vi "Spinner.vi"(5 "Enum":T1(ring)=enum."Spinner 4") -> (2 "Spinner Out":string="(---\\/------\\/---)")   [LabVIEW 2019, in "Instrument.Lockin.lvlib" / "Instrument UI.Lockin.lvclass"]
uses:
  Instrument UI.Lockin.lvclass
panel:
  in  "Spinner 6":string="(\\-\\-\\-----------)\n(-\\-\\-\\----------)\n(--\\-\\-\\---------)\n(---\\-\\-\\--------)\n(----\\-\\-\\-------)\n(-----\\-\\-\\------)\n(------\\-\\-\\-----)\n(-------\\-\\-\\----)\n(--------\\-\\-\\---)\n(---------\\-\\-\\--)\n(----------\\-\\-\\-)\n(-----------\\-\\-\\)\n(----------\\-\\-\\-)\n(---------\\-\\-\\--)\n(--------\\-\\-\\---)\n(-------\\-\\-\\----)\n(------\\-\\-\\-----)\n(-----\\-\\-\\------)\n(----\\-\\-\\-------)\n(---\\-\\-\\--------)\n(--\\-\\-\\---------)\n(-\\-\\-\\----------)"
  in  "Spinner 5":string="(\\------/\\------/)\n(-\\----/--\\----/-)\n(--\\--/----\\--/--)\n(---\\/------\\/---)\n(---/\\------/\\---)\n(--/--\\----/--\\--)\n(-/----\\--/----\\-)\n(/------\\/------\\)\n(\\------/\\------/)\n(-\\----/--\\----/-)\n(--\\--/----\\--/--)\n(---\\/------\\/---)\n(---/\\------/\\---)\n(--/--\\----/--\\--)\n(-/----\\--/----\\-)\n(/------\\/------\\)\n(-/----\\--/----\\-)\n(--/--\\----/--\\--)\n(---/\\------/\\---)\n(---\\/------\\/---)\n(--\\--/----\\--/--)\n(-\\----/--\\----/-)\n(\\------/\\------/)\n(/------\\/------\\)\n(-/----\\--/----\\-)\n(--/--\\----/--\\--)\n(---/\\------/\\---)\n(---\\/------\\/---)\n(--\\--/----\\--/--)\n(-\\----/--\\----/-)"
  in  "Spinner 4":string="(\\------/\\------/)\n(-\\----/--\\----/-)\n(--\\--/----\\--/--)\n(---\\/------\\/---)\n(---/\\------/\\---)\n(--/--\\----/--\\--)\n(-/----\\--/----\\-)\n(/------\\/------\\)"
  in  "Spinner 2":string="(\\--------------/)\n(-\\------------/-)\n(--\\----------/--)\n(---\\--------/---)\n(----\\------/----)\n(-----\\----/-----)\n(------\\--/------)\n(-------\\/-------)\n(-------/\\-------)\n(------/--\\------)\n(-----/----\\-----)\n(----/------\\----)\n(---/--------\\---)\n(--/----------\\--)\n(-/------------\\-)\n(/--------------\\)"
  in  "Spinner 1":string="(\\---------------)\n(-\\--------------)\n(--\\-------------)\n(---\\------------)\n(----\\-----------)\n(-----\\----------)\n(------\\---------)\n(-------\\--------)\n(--------\\-------)\n(---------\\------)\n(----------\\-----)\n(-----------\\----)\n(------------\\---)\n(-------------\\--)\n(--------------\\-)\n(---------------\\)\n(---------------/)\n(--------------/-)\n(-------------/--)\n(------------/---)\n(-----------/----)\n(----------/-----)\n(---------/------)\n(--------/-------)\n(-------/--------)\n(------/---------)\n(-----/----------)\n(----/-----------)\n(---/------------)\n(--/-------------)\n(-/--------------)\n(/---------------)"
  in  "spinner 3":string="(\\-\\-\\-----------)\n(-\\-\\-\\----------)\n(--\\-\\-\\---------)\n(---\\-\\-\\--------)\n(----\\-\\-\\-------)\n(-----\\-\\-\\------)\n(------\\-\\-\\-----)\n(-------\\-\\-\\----)\n(--------\\-\\-\\---)\n(---------\\-\\-\\--)\n(----------\\-\\-\\-)\n(-----------\\-\\-\\)\n(------------\\-\\/)\n(-------------\\/\\)\n(-------------/\\/)\n(------------/-/\\)\n(-----------/-/-/)\n(----------/-/-/-)\n(---------/-/-/--)\n(--------/-/-/---)\n(-------/-/-/----)\n(------/-/-/-----)\n(-----/-/-/------)\n(----/-/-/-------)\n(---/-/-/--------)\n(--/-/-/---------)\n(-/-/-/----------)\n(/-/-/-----------)\n(\\/-/------------)\n(/\\/-------------)\n(\\/\\-------------)\n(/\\-\\------------)"
  # "(\\------/\\------/)\n(-\\----/--\\----/-)\n(--\\--/----\\--/--)\n(---\\/------\\/---)\n(---/\\------/\\---)\n(--/--\\----/--\\--)\n(-/----\\--/----\\-)\n(/------\\/------\\)\n(\\------/\\------/)\n(-\\----/--\\----/-)\n(--\\--/----\\--/--)\n(---\\/------\\/---)\n(---/\\------/\\---)\n(--/--\\----/--\\--)\n(-/----\\--/----\\-)\n(/------\\/------\\)\n(-/----\\--/----\\-)\n(--/--\\----/--\\--)\n(---/\\------/\\---)\n(---\\/------\\/---)\n(--\\--/----\\--/--)\n(-\\----/--\\----/-)\n(\\------/\\------/)\n(/------\\/------\\)\n(-/----\\--/----\\-)\n(--/--\\----/--\\--)\n(---/\\------/\\---)\n(---\\/------\\/---)\n(--\\--/----\\--/--)\n(-\\----/--\\----/-)"
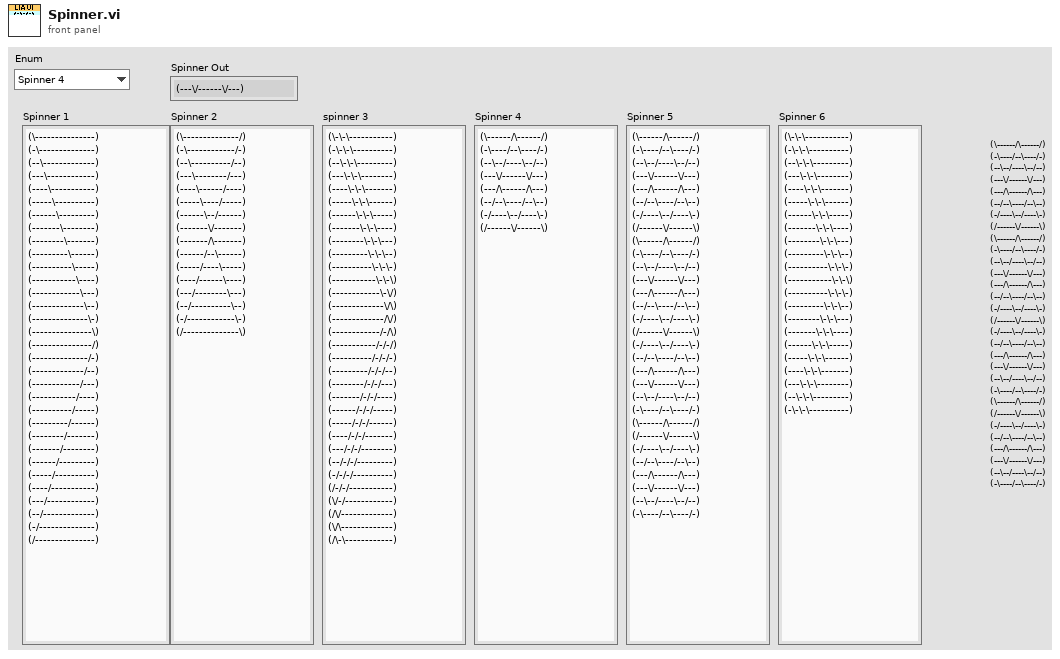
[diagram p1: front panel]
types:
  T1 = enum16{"Spinner 1", "Spinner 2", "Spinner 3", "Spinner 4", "Spinner 5", "Spinner 6"}
  T2 = enum32{"Bad", "Idle", "Run top level", "Running"}
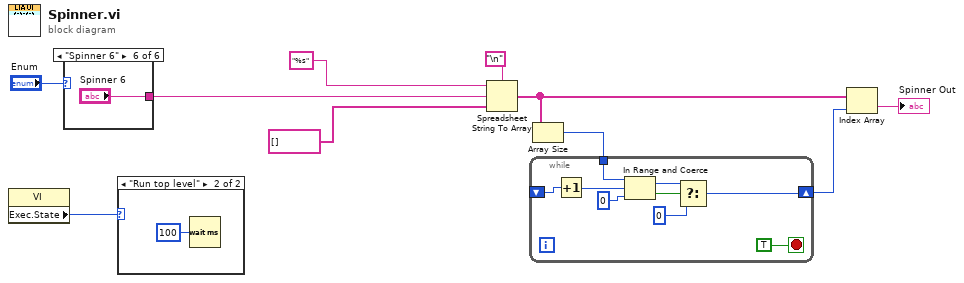
[diagram p0: block diagram]
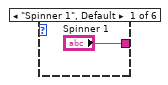
[diagram p3: hidden frame]
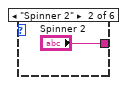
[diagram p4: hidden frame]
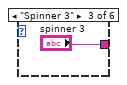
[diagram p5: hidden frame]
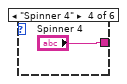
[diagram p6: hidden frame]
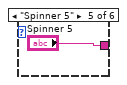
[diagram p7: hidden frame]
diagram:
  n1 = property class="VI"() -> ("Exec.State"=w2:T2)  [unwired: 2 in, 2 out]
  n2 = case shown="\"Spinner 6\"" "Enum" {
    tunnel: ["Spinner 1" "Spinner 2" "spinner 3" "Spinner 4" "Spinner 5" "Spinner 6"] -> w3
    frame "Spinner 1", Default {
    }
    frame "Spinner 2" {
    }
    frame "Spinner 3" {
    }
    frame "Spinner 4" {
    }
    frame "Spinner 5" {
    }
    frame "Spinner 6" {
    }
  }
  n3 = case shown="\"Run top level\"" w2 {
    frame Default {
    }
    frame "Run top level" {
      n4 = Wait (ms)(milliseconds to wait=u32 100) -> ()  [unwired: 1 out]
    }
  }
  n5 = Spreadsheet String To Array(delimiter (Tab)="\n", format string="%s", spreadsheet string=w3, array type (2D Dbl)=string[] []) -> (array=w7:string[])
  n6 = Array Size(array=w7) -> (size(s)=w6:i32)
  n7 = while {
    shift-right: [w20] -> w8
    shift-left: _ -> [w26]
    tunnel: w6 -> [w18]
    stop <- TRUE stop-if-true
    n8 = Increment(x=w26) -> (x+1=w22:u32)
    n9 = In Range and Coerce(upper limit=w18, x=w22, lower limit=u32 0) -> (coerced(x)=w23:u32, In Range?=w24:bool)
    n10 = Select(t=w23, s=w24, f=u32 0) -> (s? t:f=w20:u32)
  }
  n11 = Index Array(array=w7, index=w8) -> (element=→"Spinner Out":string)
